vi "To JSON.vi"(0 "Anything":variant, 1 "Pretty Print (F)":bool) -> (2 "JSON":string)   [LabVIEW 2011, in "LV JSON.lvlib"]
uses:
  LV JSON.lvlib
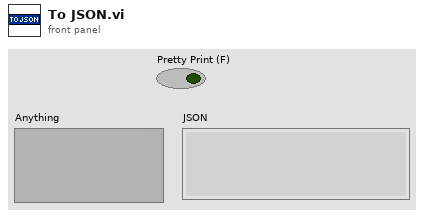
[diagram p1: front panel]
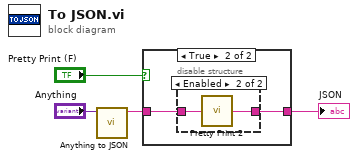
[diagram p0: block diagram]
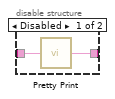
[diagram p3: hidden frame]
diagram:
  n1 = call "Anything to JSON.vi"("Anything"="Anything") -> ("JSON"=w2:string)  [unwired: 8 in, 2 out]
  n2 = case shown="True" "Pretty Print (F)" {
    tunnel: w2 -> [w5 w7]
    tunnel: [w5 w6] -> w1
    frame False {
    }
    frame True {
      n3 = disable-structure shown="Enabled" {
        disable-tunnel: w7 -> [w9 w11]
        disable-tunnel: [w8 w10] -> w6
        frame Disabled {
          n4 = call "Pretty Print.vi"("JSON String"=w9) -> ("Pretty JSON String"=w8:string)  [unwired: 1 out]
        }
        frame Enabled {
          n5 = call "Pretty Print 2.vi"("JSON String"=w11) -> ("Pretty JSON String"=w10:string)  [unwired: 1 out]
        }
      }
    }
  }
  "JSON" <- w1
